vi "VIH UI - Insert HTML Tag to String.vi"(6 "cmd":enum32{"nop", "<a>", "<b>", "<i>", "<u>"}(ring), 8 "tag 2":string, 9 "tag 1":string, 10 "Project Tree":T1, 11 "Str Refnum":refnum<vi>) -> (3 "dup Str Refnum":refnum<vi>)   [LabVIEW 2014]
doc: "::: VI Helpeks :::\nCopyright (c) 2000-2026 Konstantin Shifershteyn. All rights reserved."
uses:
  VIH Project Tree Typedef - Tree Refnum.ctl
panel:
  # "VI Helpeks\nCopyright (c) 2012-2026 Konstantin Shifershteyn"
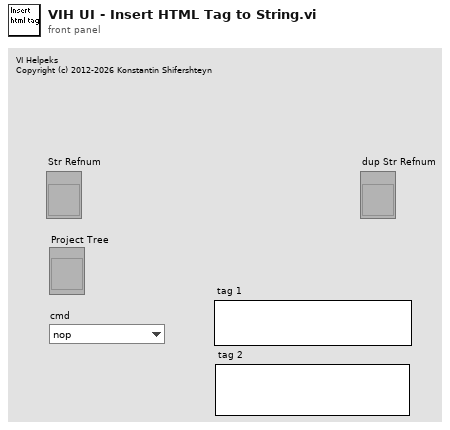
[diagram p1: front panel]
types:
  T1 = typedef "VIH Project Tree Typedef - Tree Refnum.ctl" = refnum<vi>
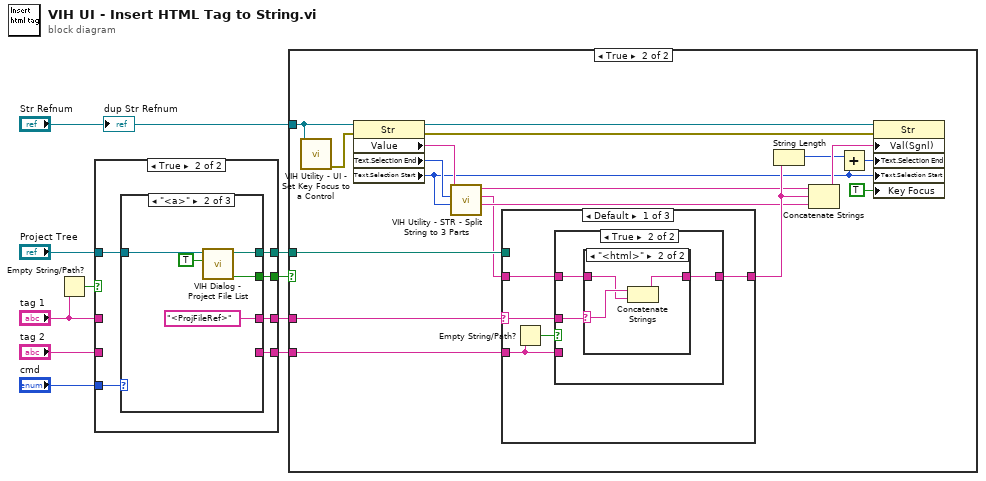
[diagram p0: block diagram]
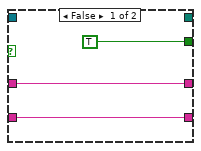
[diagram p2: hidden frame]
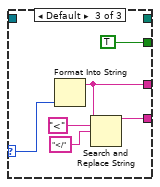
[diagram p4: hidden frame]
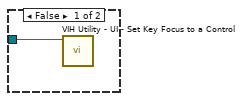
[diagram p5: hidden frame]
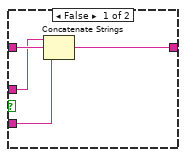
[diagram p6: hidden frame]
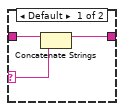
[diagram p7: hidden frame]
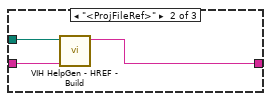
[diagram p8: hidden frame]
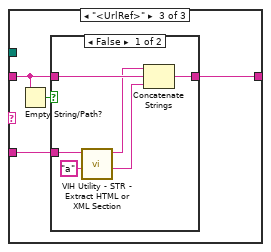
[diagram p9: hidden frame]
diagram:
  n1 = Empty String/Path?(string/path="tag 1") -> (empty?=w6:bool)
  n2 = case shown="True" w6 {
    tunnel: [_ w19] -> w10
    tunnel: [TRUE w18] -> w9
    tunnel: "Project Tree" -> [_ w17]
    tunnel: "cmd" -> [_ w16]
    tunnel: [w13 w15] -> w5
    tunnel: "tag 1" -> [w13 _]
    tunnel: [w12 w14] -> w3
    tunnel: "tag 2" -> [w12 _]
    frame False {
    }
    frame True {
      n3 = case shown="\"<a>\"" w16 {
        selector: w16 -> [_ _ w26]
        tunnel: [_ w24 _] -> w19
        tunnel: [_ w23 TRUE] -> w18
        tunnel: w17 -> [_ w22 _]
        tunnel: [_ "<ProjFileRef>" w27] -> w15
        tunnel: [_ _ w25] -> w14
        frame "nop" {
        }
        frame "<a>" {
          n4 = call "VIH Dialog - Project File List.vi"("Disable not buildable"=TRUE, "Project Tree"=w22) -> ("OK out"=w23:bool, "File Path"=w24:path)  [unwired: 7 in, 1 out]
        }
        frame Default {
          n5 = Format Into String(w26) -> (resulting string=w27:string)  [unwired: 3 in, 1 out]
          n6 = Search and Replace String(input string=w27, search string="<", replace string="</" ("search string")) -> (result string=w25:string)  [unwired: 5 in, 3 out]
        }
      }
    }
  }
  n7 = case shown="True" w9 {
    tunnel: w10 -> [_ w45]
    tunnel: "Str Refnum" -> [w31 w43]
    tunnel: w5 -> [_ w33]
    tunnel: w3 -> [_ w32]
    frame False {
      n8 = call "VIH Utility - UI - Set Key Focus to a Control.vi"("Ctl Refnum"=w31) -> ()  [unwired: 9 in, 2 out]
    }
    frame True {
      n9 = call "VIH Utility - UI - Set Key Focus to a Control.vi"("Ctl Refnum"=w43) -> ("error out"=w46:errorcluster)  [unwired: 9 in, 1 out]
      n10 = property on="Property Node" class="Str"(reference=w43, error in=w46) -> (reference out=w42:refnum<vi>, error out=w41:errorcluster, "Value"=w39:string, "Text.Selection End"=w38:u32, "Text.Selection Start"=w37:u32)
      n11 = call "VIH Utility - STR - Split String to 3 Parts.vi"("Position 2"=w37, "Position 1"=w38, "String"=w39) -> ("After"=w35:string, "Middle"=w34:string, "Before"=w36:string)  [unwired: 6 in]
      n12 = case shown="Default" w33 {
        selector: w33 -> [w52 _ _]
        tunnel: w45 -> [_ w70 _]
        tunnel: [w53 w69 w73] -> w44
        tunnel: w34 -> [w51 w68 w71]
        tunnel: w32 -> [w50 _ w72]
        frame Default {
          n13 = Empty String/Path?(string/path=w50) -> (empty?=w54:bool)
          n14 = case shown="True" w54 {
            tunnel: [w57 w61] -> w53
            tunnel: w52 -> [w56 w59]
            tunnel: w51 -> [w58 w60]
            tunnel: w50 -> [w55 _]
            frame False {
              n15 = Concatenate Strings(w56, w58, w55) -> (w57:string)
            }
            frame True {
              n16 = case shown="\"<html>\"" w59 {
                selector: w59 -> [w62 w67]
                tunnel: [w64 w65] -> w61
                tunnel: w60 -> [w63 w66]
                frame Default {
                  n17 = Concatenate Strings(w63, w62) -> (w64:string)
                }
                frame "<html>" {
                  n18 = Concatenate Strings(w67, w66) -> (w65:string)
                }
              }
            }
          }
        }
        frame "<ProjFileRef>" {
          n19 = call "VIH HelpGen - HREF - Build.vi"("Text to enclose"=w68, "File Path"=w70) -> ("A HREF"=w69:string)  [unwired: 9 in]
        }
        frame "<UrlRef>" {
          n20 = Empty String/Path?(string/path=w71) -> (empty?=w74:bool)
          n21 = case shown="False" w74 {
            tunnel: [w77 w81] -> w73
            tunnel: w72 -> [w80 w81]
            tunnel: w71 -> [w78 _]
            frame False {
              n22 = call "VIH Utility - STR - Extract HTML or XML Section.vi"("Section name"="a", "HTML in"=w80) -> ("end"=w75:string, "start"=w76:string)  [unwired: 5 in, 3 out]
              n23 = Concatenate Strings(w76, w78, w75) -> (w77:string)
            }
            frame True {
            }
          }
        }
      }
      n24 = String Length(string=w44) -> (length=w40:i32)
      n25 = Concatenate Strings(w36, w44, w35) -> (w47:string)
      n26 = Add(x=w40, y=w37) -> (x+y=w48:u32)
      n27 = property on="Property Node" class="Str"(reference=w42, error in=w41, "Val(Sgnl)"=w47, "Text.Selection End"=w48, "Text.Selection Start"=w37, "Key Focus"=TRUE) -> ()  [unwired: 2 out]
    }
  }
  "dup Str Refnum" <- "Str Refnum"
